vi "View TDMS.vi"() -> ()   [LabVIEW 2026]
panel:
  out "Waveform Graph":waveform(dbl)[](graph)
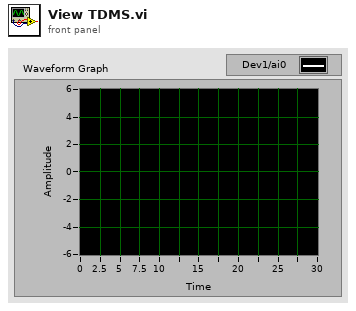
[diagram p1: front panel]
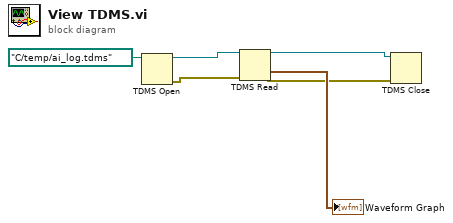
[diagram p0: block diagram]
diagram:
  n1 = TDMS Open(11:path "C:/temp/ai_log.tdms" ("file path")) -> (0:w4:errorcluster, 3:w5:refnum<k34>)  [unwired: 6 in]
  n2 = TDMS Read(0:w5, 11:w4) -> (4:w2:refnum<k34>, 10:→"Waveform Graph":waveform(dbl)[], 15:w1:errorcluster)  [unwired: 6 in, 3 out]
  n3 = TDMS Close(8:w1, 11:w2) -> ()  [unwired: 2 out]
